vi "Save Item.vi"(8 "error in (no error)":errorcluster, 10 "Save Icon?":bool, 11 "VI in":refnum<class "VI.lvclass">) -> (0 "error out":errorcluster, 2 "Saved?":bool, 3 "VI out":refnum<class "VI.lvclass">)   [LabVIEW 2020, in "VI Properties Editor.lvlib" / "VI.lvclass"]
doc: "Saves the new data of <B>VI in</B>."
uses:
  VI.lvclass
  Control/Control.lvclass
  <vilib>/LabVIEW Icon API/lv_icon/Classes/Icon/Icon.lvclass
  VI.lvclass/VI.ctl
  <vilib>/LabVIEW Icon API/LabVIEW Icon API.lvlib
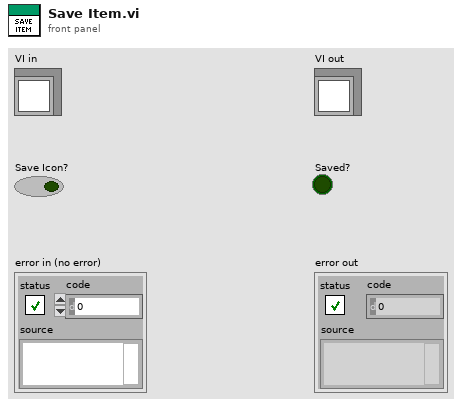
[diagram p1: front panel]
types:
  T1 = enum32{"invalid VI type", "Standard VI", "Control VI", "Global VI", "Polymorphic VI", "Configuration VI", "SubSystem", "Facade VI", "Method VI", "Statechart Diagram VI"}
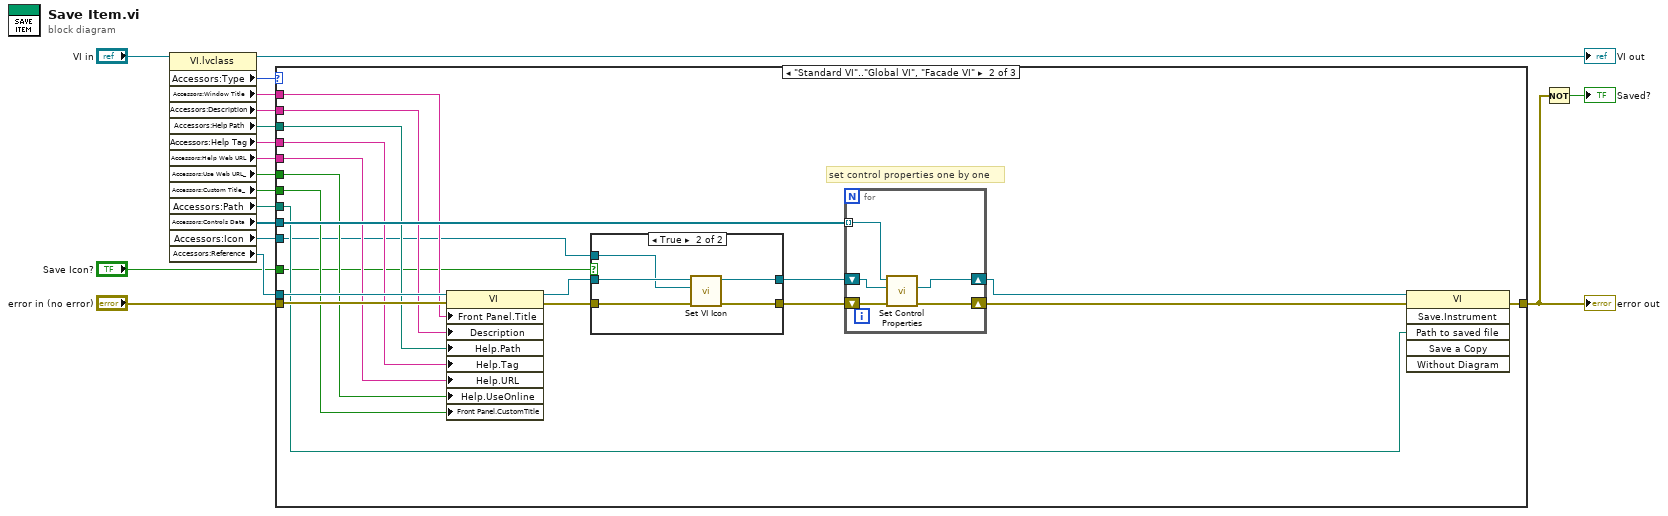
[diagram p0: block diagram]
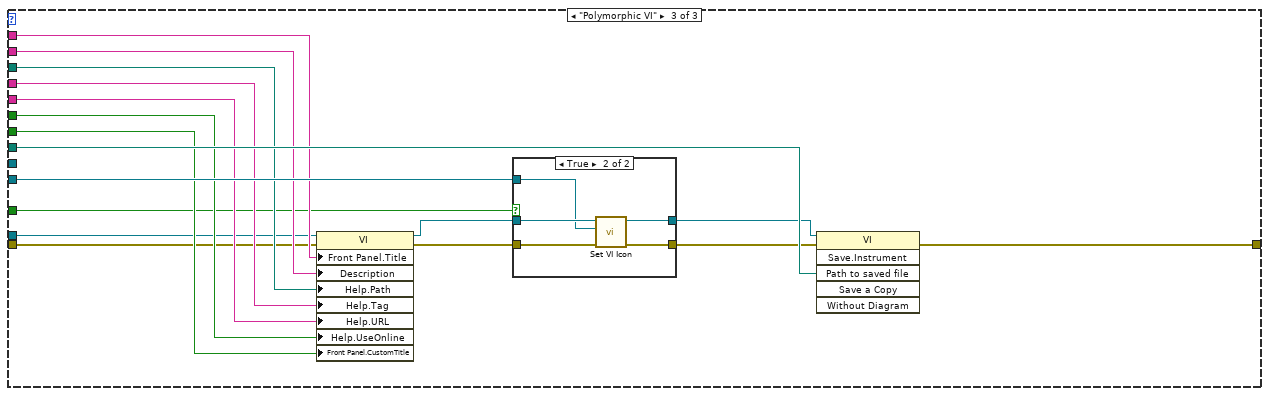
[diagram p4: hidden frame]
diagram:
  n1 = property class="VI.lvclass"(reference="VI in") -> (reference out=→"VI out":refnum<class "VI.lvclass">, "Accessors:Type"=w14:T1, "Accessors:Window Title"=w13:string, "Accessors:Description"=w12:string, "Accessors:Help Path"=w11:path, "Accessors:Help Tag"=w10:string, "Accessors:Help Web URL"=w9:string, "Accessors:Use Web URL_"=w8:bool, "Accessors:Custom Title_"=w7:bool, "Accessors:Path"=w6:path, "Accessors:Controls Data"=w5:refnum<class "Control.lvclass">[], "Accessors:Icon"=w2:refnum<class "Icon.lvclass">, "Accessors:Reference"=w4:refnum<vi>)  [unwired: 1 in, 1 out]
  n2 = case shown="\"Standard VI\"..\"Global VI\", \"Facade VI\"" w14 {
    tunnel: [w19 w39 w66] -> w18
    tunnel: w4 -> [_ w35 w55]
    tunnel: "error in (no error)" -> [w19 w37 w56]
    tunnel: w12 -> [_ w33 w61]
    tunnel: w10 -> [_ w31 w62]
    tunnel: w11 -> [_ w30 w63]
    tunnel: w6 -> [_ w29 w65]
    tunnel: w5 -> [_ w34 _]
    tunnel: w13 -> [_ w32 w60]
    tunnel: w7 -> [_ w28 w64]
    tunnel: w9 -> [_ w27 w59]
    tunnel: w8 -> [_ w26 w58]
    tunnel: w2 -> [_ w24 w67]
    tunnel: "Save Icon?" -> [_ w20 w52]
    frame "invalid VI type", Default {
    }
    frame "Standard VI".."Global VI", "Facade VI" {
      # "set control properties one by one"
      n3 = property class="VI"(reference=w35, error in=w37, "Front Panel.Title"=w32, "Description"=w33, "Help.Path"=w30, "Help.Tag"=w31, "Help.URL"=w27, "Help.UseOnline"=w26, "Front Panel.CustomTitle"=w28) -> (reference out=w25:refnum<vi>, error out=w36:errorcluster)
      n4 = case shown="True" w20 {
        tunnel: w36 -> [w40 w46]
        tunnel: w25 -> [w41 w45]
        tunnel: w24 -> [_ w44]
        tunnel: [w40 w43] -> w23
        tunnel: [w41 w42] -> w22
        frame False {
        }
        frame True {
          n5 = call <vilib>:"Set VI Icon.vi"("error in (no error)"=w46, "Icon"=w44, "VI Refnum in"=w45) -> ("error out"=w43:errorcluster, "VI Refnum out"=w42:refnum<vi>)  [unwired: 7 in]
        }
      }
      n6 = for {
        shift-right: [w47] -> w38
        shift-left: w23 -> [w51]
        tunnel: w34 -> [w49] mode=indexing
        shift-right: [w48] -> w21
        shift-left: w22 -> [w50]
        n7 = call-dynamic "Set Control Properties.vi"("error in (no error)"=w51, "Owning VI"=w50, "Control in"=w49) -> ("error out"=w47:errorcluster, "dup Owning VI"=w48:refnum<vi>)  [unwired: 6 in, 1 out]
      }
      n8 = invoke class="VI" method="Save.Instrument"(reference=w21, error in=w38, "Path to saved file"=w29) -> (error out=w39:errorcluster)  [unwired: 3 in, 5 out]
    }
    frame "Polymorphic VI" {
      n9 = property class="VI"(reference=w55, error in=w56, "Front Panel.Title"=w60, "Description"=w61, "Help.Path"=w63, "Help.Tag"=w62, "Help.URL"=w59, "Help.UseOnline"=w58, "Front Panel.CustomTitle"=w64) -> (reference out=w68:refnum<vi>, error out=w57:errorcluster)
      n10 = case shown="True" w52 {
        tunnel: w68 -> [w70 w75]
        tunnel: w67 -> [_ w74]
        tunnel: w57 -> [w69 w73]
        tunnel: [w69 w72] -> w54
        tunnel: [w70 w71] -> w53
        frame False {
        }
        frame True {
          n11 = call <vilib>:"Set VI Icon.vi"("error in (no error)"=w73, "Icon"=w74, "VI Refnum in"=w75) -> ("error out"=w72:errorcluster, "VI Refnum out"=w71:refnum<vi>)  [unwired: 7 in]
        }
      }
      n12 = invoke class="VI" method="Save.Instrument"(reference=w53, error in=w54, "Path to saved file"=w65) -> (error out=w66:errorcluster)  [unwired: 3 in, 5 out]
    }
  }
  "error out" <- w18
  n13 = Not(x=w18) -> (.not. x?=→"Saved?":bool)
